vi "Write VISA resource name.vi"(8 "error in (no error)":errorcluster, 10 "VISA resource name":refnum<visa-resource-name>, 11 "CTI_Bus in":refnum<class "CTI_Bus.lvclass">) -> (0 "error out":errorcluster, 3 "CTI_Bus out":refnum<class "CTI_Bus.lvclass">)   [LabVIEW 2021, in "CTI_Bus.lvclass"]
uses:
  CTI_Bus.lvclass
  CTI_Bus.lvclass/CTI_Bus.ctl
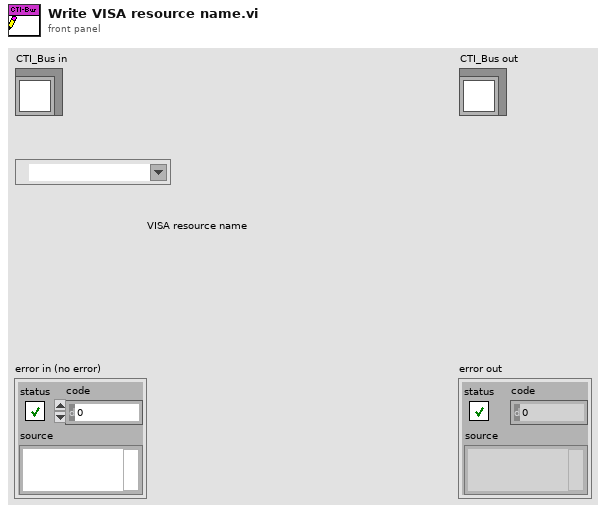
[diagram p1: front panel]
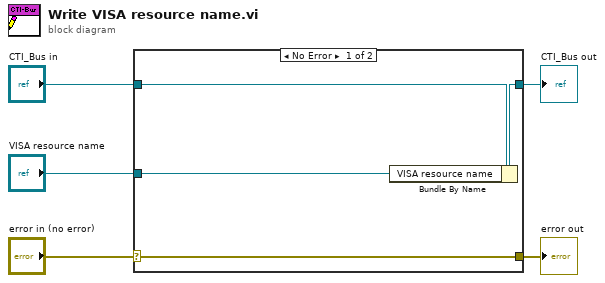
[diagram p0: block diagram]
diagram:
  n1 = case shown="No Error" "error in (no error)" {
    selector: "error in (no error)" -> [w9 w10]
    tunnel: [w9 w10] -> w4
    tunnel: [w7 w11] -> w2
    tunnel: "CTI_Bus in" -> [w8 w11]
    tunnel: "VISA resource name" -> [w6 _]
    frame No Error {
      n2 = Bundle By Name(cluster=w8, "VISA resource name"=w6) -> (w7:refnum<class "CTI_Bus.lvclass">)
    }
    frame Error {
    }
  }
  "error out" <- w4
  "CTI_Bus out" <- w2
